vi "Run UI Support Tests.vi"(8 "error in":errorcluster, 11 "Work Folder":path) -> (0 "error out":errorcluster, 2 "Report":string, 3 "All Passed":bool)   [LabVIEW 2026]
doc: "Runs every UI Support test VI (Tests\\UI Support) and reports one overall result. Test Data Folder is Tests\\Storage\\Test Data next to this VI; each test copies what it needs from there into a new case folder under Work Folder, so the tests can be repeated and never touch the real data in %LOCALAPPDATA%\\LVTimeTracker. An empty Work Folder (or Not a Path) means the system temp folder, in a subfolder named LVTimeTracker Tests.\n\nInputs: Work Folder; error in. Outputs: All Passed (TRUE only when every test passed); Report (every check of every test, one section per test); error out (every test's error, merged).\n\nGenerated by: Claude"
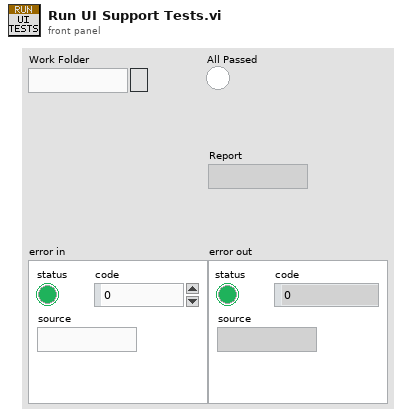
[diagram p1: front panel]
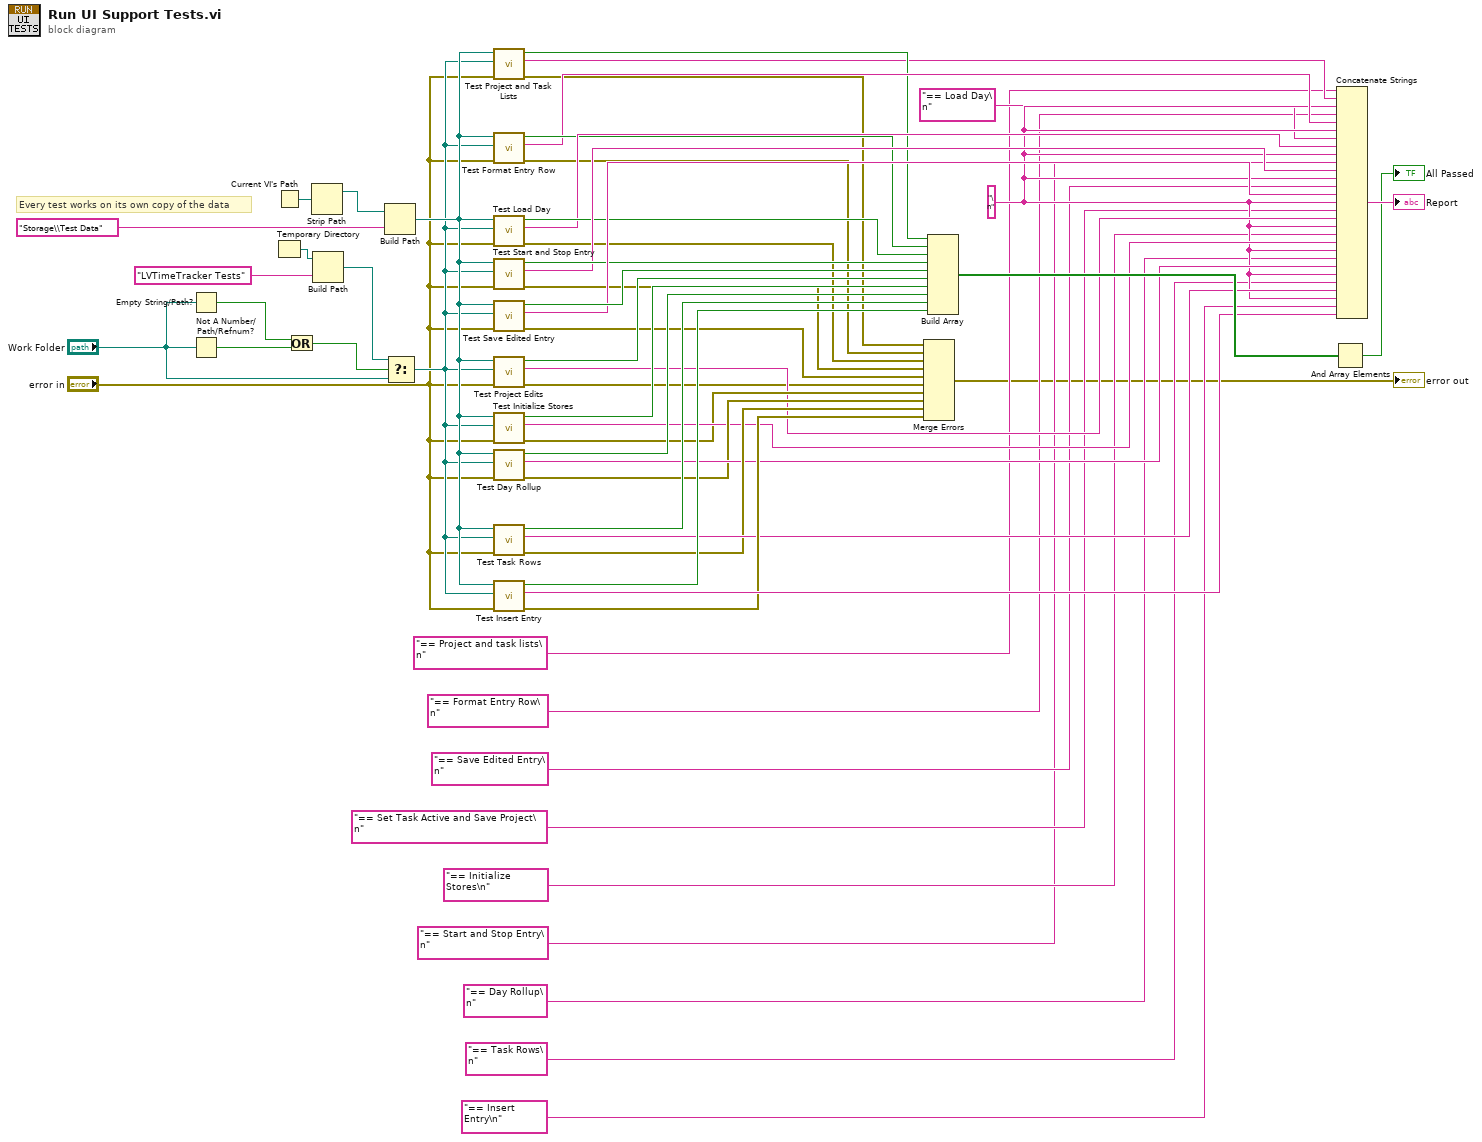
[diagram p0: block diagram]
diagram:
  w18 = "\n" ("newline")
  # "Every test works on its own copy of the data"
  n1 = Empty String/Path?(string/path="Work Folder") -> (empty?=w20:bool)
  n2 = Not A Number/Path/Refnum?(number/path/refnum="Work Folder") -> (NaN/Path/Refnum?=w21:bool)
  n3 = Temporary Directory() -> (w19:path)
  n4 = Current VI's Path() -> (path=w22:path)
  n5 = Or(x=w20, y=w21) -> (x .or. y?=w24:bool)
  n6 = Strip Path(path=w22) -> (stripped path=w25:path)  [unwired: 1 out]
  n7 = Build Path(base path=w19, name or relative path="LVTimeTracker Tests" ("temp subfolder")) -> (appended path=w23:path)
  n8 = Build Path(base path=w25, name or relative path="Storage\\Test Data" ("test data")) -> (appended path=w27:path)
  n9 = Select(t=w23, s=w24, f="Work Folder") -> (s? t:f=w26:path)
  n10 = call "Test Project and Task Lists.vi"("error in"="error in", "Work Folder"=w26, "Test Data Folder"=w27) -> ("error out"=w28:errorcluster, "Report"=w29:string, "Passed"=w30:bool)  [unwired: 6 in]
  n11 = call "Test Format Entry Row.vi"("error in"="error in", "Work Folder"=w26, "Test Data Folder"=w27) -> ("error out"=w31:errorcluster, "Report"=w32:string, "Passed"=w33:bool)  [unwired: 6 in]
  n12 = call "Test Load Day.vi"("error in"="error in", "Work Folder"=w26, "Test Data Folder"=w27) -> ("error out"=w34:errorcluster, "Report"=w35:string, "Passed"=w36:bool)  [unwired: 6 in]
  n13 = call "Test Start and Stop Entry.vi"("error in"="error in", "Work Folder"=w26, "Test Data Folder"=w27) -> ("error out"=w37:errorcluster, "Report"=w38:string, "Passed"=w39:bool)  [unwired: 6 in]
  n14 = call "Test Save Edited Entry.vi"("error in"="error in", "Work Folder"=w26, "Test Data Folder"=w27) -> ("error out"=w40:errorcluster, "Report"=w41:string, "Passed"=w42:bool)  [unwired: 6 in]
  n15 = call "Test Project Edits.vi"("error in"="error in", "Work Folder"=w26, "Test Data Folder"=w27) -> ("error out"=w43:errorcluster, "Report"=w44:string, "Passed"=w45:bool)  [unwired: 6 in]
  n16 = call "Test Initialize Stores.vi"("error in"="error in", "Work Folder"=w26, "Test Data Folder"=w27) -> ("error out"=w46:errorcluster, "Report"=w47:string, "Passed"=w48:bool)  [unwired: 6 in]
  n17 = call "Test Day Rollup.vi"("error in"="error in", "Work Folder"=w26, "Test Data Folder"=w27) -> ("error out"=w49:errorcluster, "Report"=w50:string, "Passed"=w51:bool)  [unwired: 6 in]
  n18 = call "Test Task Rows.vi"("error in"="error in", "Work Folder"=w26, "Test Data Folder"=w27) -> ("error out"=w52:errorcluster, "Report"=w53:string, "Passed"=w54:bool)  [unwired: 6 in]
  n19 = call "Test Insert Entry.vi"("error in"="error in", "Work Folder"=w26, "Test Data Folder"=w27) -> ("error out"=w55:errorcluster, "Report"=w56:string, "Passed"=w57:bool)  [unwired: 6 in]
  n20 = Merge Errors(w28, w31, w34, w37, w40, w43, w46, w49, w52, w55) -> (→"error out":errorcluster)
  n21 = Build Array(w30, w33, w36, w39, w42, w45, w48, w51, w54, w57) -> (w58:bool[])
  n22 = And Array Elements(Boolean array=w58) -> (logical AND=→"All Passed":bool)
  n23 = Concatenate Strings("== Project and task lists\n" ("h1"), w29, w18, "== Format Entry Row\n" ("h2"), w32, w18, "== Load Day\n" ("h3"), w35, w18, "== Start and Stop Entry\n" ("h4"), w38, w18, "== Save Edited Entry\n" ("h5"), w41, w18, "== Set Task Active and Save Project\n" ("h6"), w44, w18, "== Initialize Stores\n" ("h7"), w47, w18, "== Day Rollup\n" ("h8"), w50, w18, "== Task Rows\n" ("h9"), w53, w18, "== Insert Entry\n" ("h10"), w56) -> (→"Report":string)
